vi "Add Bitfile Dependency.vi"(8 "error in (no error)":errorcluster, 10 "Path":path, 11 "Item Ref in":T1 format="%.0x") -> (0 "error out":errorcluster, 2 "bitfile changed":bool, 3 "Item Ref out":T1 format="%.0x")   [LabVIEW 2020, in "FPGA Addon System Explorer.lvlib"]
uses:
  FPGA Addon System Explorer.lvlib
  <vilib>/NI VeriStand/Custom Device API/Custom Device Item Ref.ctl
  <vilib>/NI VeriStand/Custom Device API/Dependent File Optional Info.ctl
  Addon Shared/SubVIs/Constants.vi
  <vilib>/NI VeriStand/Custom Device API/Get Item Property (Dependent File).vi
  <vilib>/NI VeriStand/Custom Device API/Set Item Property (Dependent File).vi
  <vilib>/NI VeriStand/Custom Device API/Custom Device API.lvlib
  Addon Shared/FPGA Addon Shared.lvlib
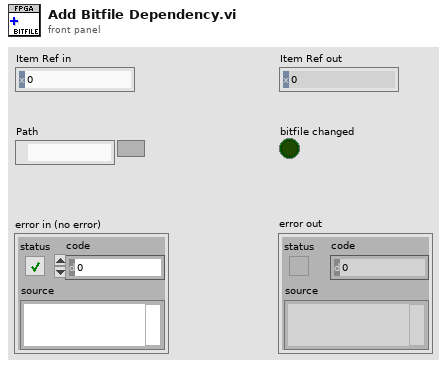
[diagram p1: front panel]
types:
  T1 = typedef "Custom Device API.lvlib/Custom Device Item Ref.ctl" = u64
  T2 = typedef "Custom Device API.lvlib/Dependent File Optional Info.ctl" = cluster{"Version":string, "RTDestination":path, "ForceDownload":bool, "SupportedTarget":string, "MD5":string}
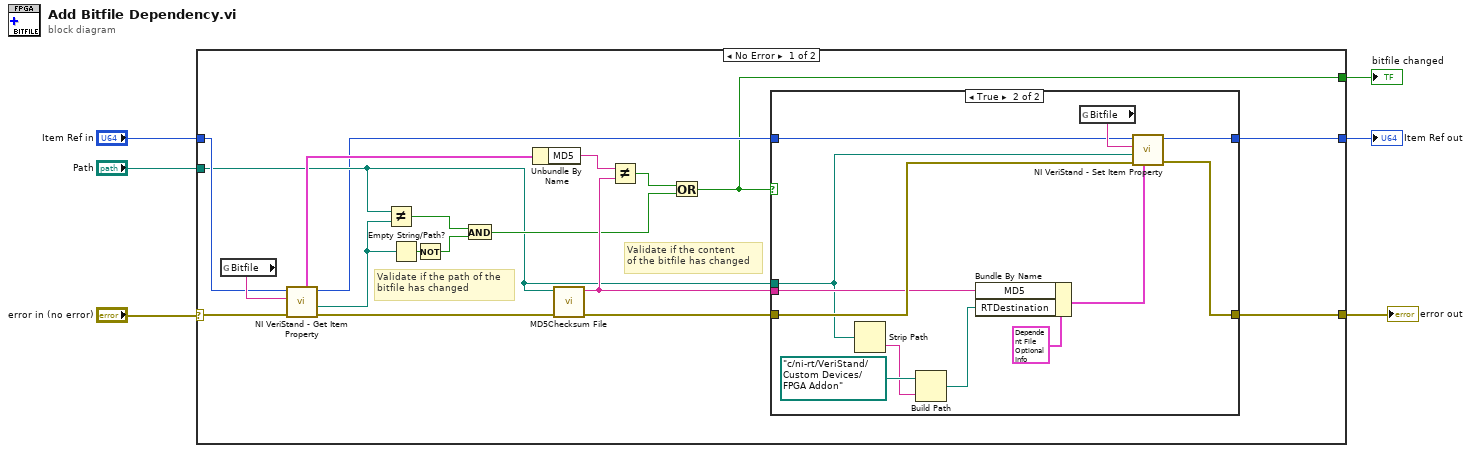
[diagram p0: block diagram]
diagram:
  n1 = case shown="No Error" "error in (no error)" {
    selector: "error in (no error)" -> [w20 w41]
    tunnel: "Item Ref in" -> [w21 w40]
    tunnel: [w24 w41] -> w5
    tunnel: [w23 w40] -> w4
    tunnel: "Path" -> [w9 _]
    tunnel: [w7 _] -> w1
    frame No Error {
      # "Validate if the path of the \nbitfile has changed"
      # "Validate if the content \nof the bitfile has changed"
      n2 = global read "Constants.vi" "Bitfile"() -> (w22:string)
      n3 = call-poly <vilib>:"NI VeriStand - Get Item Property.vi"("error in (no error)"=w20, "Property Name"=w22, "Item Ref in"=w21) -> ("error out"=w18:errorcluster, "Path"=w12:path, "Item Ref out"=w8:T1, "OptionalInfo"=w19:T2)  [unwired: 4 in, 1 out]
      n4 = Not Equal?(x=w9, y=w12) -> (x != y?=w15:bool)
      n5 = Empty String/Path?(string/path=w12) -> (empty?=w13:bool)
      n6 = Not(x=w13) -> (.not. x?=w14:bool)
      n7 = And(x=w15, y=w14) -> (x .and. y?=w10:bool)
      n8 = Unbundle By Name(w19) -> ("MD5"=w17:string)
      n9 = call <vilib>:"MD5Checksum File.vi"("error in (no error)"=w18, "Path"=w9) -> ("error out"=w25:errorcluster, "MD5 message-digest"=w16:string)  [unwired: 8 in]
      n10 = Not Equal?(x=w17, y=w16) -> (x != y?=w11:bool)
      n11 = Or(x=w11, y=w10) -> (x .or. y?=w7:bool)
      n12 = case shown="True" w7 {
        tunnel: w25 -> [w26 w39]
        tunnel: [w26 w36] -> w24
        tunnel: [w27 w35] -> w23
        tunnel: w16 -> [_ w30]
        tunnel: w9 -> [_ w29]
        tunnel: w8 -> [w27 w28]
        frame False {
        }
        frame True {
          n13 = Strip Path(path=w29) -> (name=w32:string)  [unwired: 1 out]
          n14 = Build Path(base path=path "c:/ni-rt/VeriStand/Custom Devices/FPGA Addon" ("RTDestination"), name or relative path=w32) -> (appended path=w31:path)
          n15 = Bundle By Name(cluster=T2 {"Version"="1.0", "RTDestination"=path "c:/ni-rt/VeriStand/Custom Devices/FPGA Addon", "ForceDownload"=FALSE, "SupportedTarget"="All", "MD5"=""} ("OptionalInfo"), "MD5"=w30, "RTDestination"=w31) -> (w38:T2)
          n16 = global read "Constants.vi" "Bitfile"() -> (w34:string)
          n17 = call-poly <vilib>:"NI VeriStand - Set Item Property.vi"("OptionalInfo"=w38, "error in (no error)"=w39, "Path"=w29, "Property Name"=w34, "Item Ref in"=w28) -> ("error out"=w36:errorcluster, "Item Ref out"=w35:T1)  [unwired: 4 in, 1 out]
        }
      }
    }
    frame Error {
    }
  }
  "error out" <- w5
  "Item Ref out" <- w4
  "bitfile changed" <- w1
